vi "Read localPort.vi"(8 "error in (no error)":errorcluster, 11 "ZM-CP-UDP-receiver in":refnum<class "ZM-CP-UDP-receiver.lvclass">) -> (0 "error out":errorcluster, 2 "localPort":u16=61557, 3 "ZM-CP-UDP-receiver out":refnum<class "ZM-CP-UDP-receiver.lvclass">)   [LabVIEW 2020, in "ZM-CP-UDP-udp_transport.lvlib" / "ZM-CP-UDP-receiver.lvclass"]
doc: "Reads one field of this class's private data. Generated by lvai_create_accessors from the class private data control."
uses:
  ZM-CP-UDP-receiver.lvclass
  ZM-CP-UDP-receiver.lvclass/ZM-CP-UDP-receiver.ctl
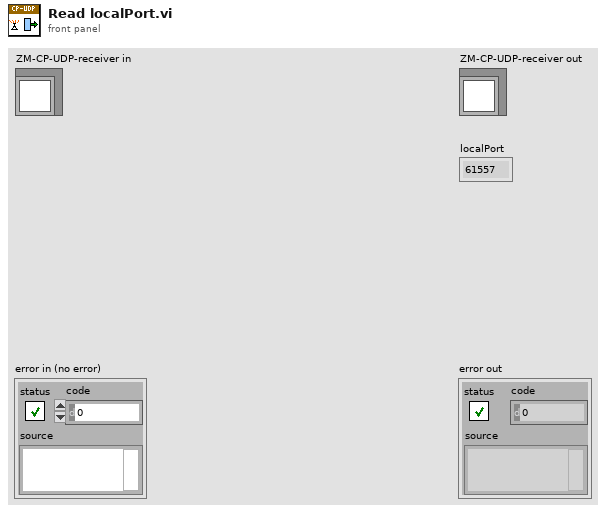
[diagram p1: front panel]
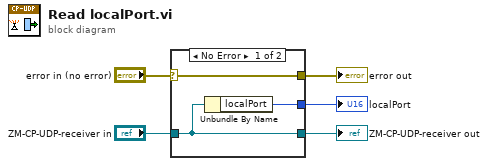
[diagram p0: block diagram]
diagram:
  n1 = case shown="No Error" "error in (no error)" {
    selector: "error in (no error)" -> [w8 w9]
    tunnel: [w8 w9] -> w4
    tunnel: [w7 w10] -> w2
    tunnel: "ZM-CP-UDP-receiver in" -> [w7 w10]
    tunnel: [w6 _] -> w1
    frame No Error {
      n2 = Unbundle By Name(w7) -> ("localPort"=w6:u16)
    }
    frame Error {
    }
  }
  "error out" <- w4
  "ZM-CP-UDP-receiver out" <- w2
  "localPort" <- w1
